vi "GetWindowTextW Wrapper Template.vi"(0 "hWnd":u64, 5 "nMaxCount":i32=256, 11 "error in":errorcluster) -> (4 "text":u16[](array[numeric]), 6 "return value":i32, 15 "error out":errorcluster)   [LabVIEW 2020]
doc: "Returns the caption of the window hWnd through user32.dll GetWindowTextW (stdcall, called in any thread) as UTF-16 code units, so a caption in any language survives (narrowing it to LabVIEW bytes would not). The buffer is nMaxCount code units of zeros, and the caption is cut at its terminating 0. For a window of LabVIEW's own process the function sends WM_GETTEXT, which LabVIEW answers also while a dialog's modal loop runs (measured on LabVIEW 2025). return value is the number of characters copied, 0 for an empty caption or on failure. When error in carries an error the DLL is not called. Generated by scripts\\Build Win32 Wrappers.vi - do not edit by hand, rebuild it."
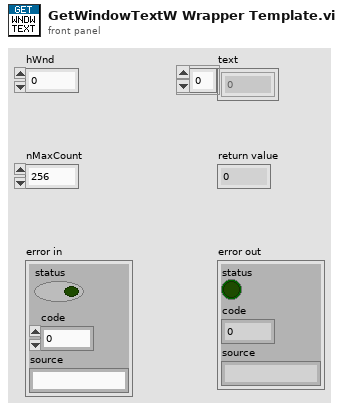
[diagram p1: front panel]
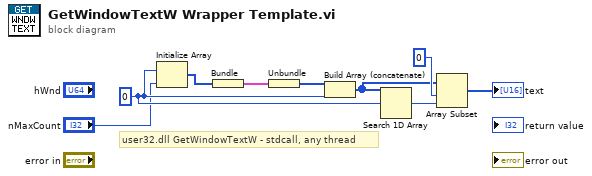
[diagram p0: block diagram]
diagram:
  w3 = u16 0
  # "user32.dll GetWindowTextW - stdcall, any thread"
  n1 = Initialize Array(w3, "nMaxCount") -> (w4:u16[])
  n2 = Bundle(w4) -> (w5:cluster{u16[]})  [unwired: 1 in]
  n3 = Unbundle(w5) -> (w6:u16[])
  n4 = Build Array (concatenate)(w6, w3) -> (w7:u16[])
  n5 = Search 1D Array(1D array=w7, element=w3) -> (index of element=w8:i32)  [unwired: 1 in]
  n6 = Array Subset(array=w7, index=0, length=w8) -> (→"text":u16[])
